vi "Read.vi"(8 "error in (no error)":errorcluster, 9 "timeout (ms)":i32=200, 10 "number to read":i32=100, 11 "CAN RW CANsub in":refnum<class "CAN RW CANsub.lvclass">) -> (0 "error out":errorcluster, 1 "Timeout":bool, 2 "pcap CAN Data":u8[](array[numeric]), 3 "CAN RW CANsub out":refnum<class "CAN RW CANsub.lvclass">, 4 "number read":i32=100)   [LabVIEW 2021, in "CAN RW CANsub.lvclass"]
doc: "Returns pcap CAN packets for at most number to read frames. Reads the socket only when no frames remain from the last read; the socket read waits at most timeout (ms). Applies the allow and deny lists. Timeout is True when no packet is returned and there is no error. Allocates the output array on each call (the interface of CAN_RW_CORE requires it)."
uses:
  CAN RW CANsub.lvclass
  C:/Program Files/National Instruments/LabVIEW 2025/vi.lib/CIF Foundation/CIF CAN RW Core/CAN_RW_CORE.lvclass
  CAN RW CANsub.lvclass/CAN RW CANsub.ctl
  <vilib>/CIF Foundation/CIF CAN RW Core/CAN_RW_CORE.lvclass/CAN_RW_CORE.ctl
  CANsub/c_client/api/CANsub_Channel/CANsub_Channel.lvclass
  CANsub/c_client/api/CANsub_API.lvlib
  <vilib>/CIF Foundation/CIF CAN RW Core/CAN_RW_CORE.lvclass
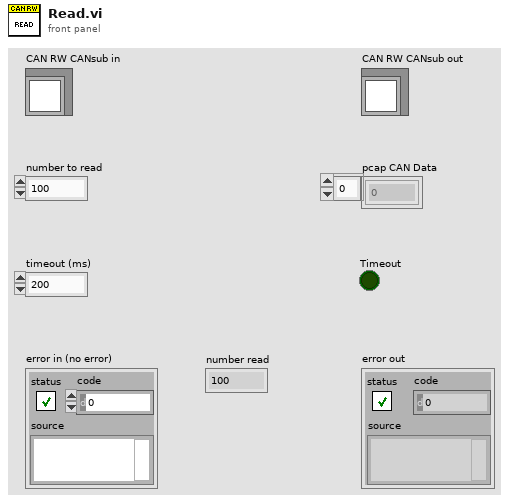
[diagram p1: front panel]
types:
  T1 = typedef "CANsub_API.lvlib/CANsub_Frames.ctl" = cluster{"count":i32, "t_dev":dbl[], "id":u32[], "flags":u16[], "dlc":u8[], "data len":u8[], "data":u8[]}
  T2 = typedef "CANsub_API.lvlib/CANsub_Pcap_Options.ctl" = cluster{"allow list":u32[], "deny list":u32[], "TAI minus UTC (s)":i32, "keep TX acks":bool, "little endian":bool}
  T3 = typedef "CANsub_API.lvlib/CANsub_Pcap_Results.ctl" = cluster{"length":i32, "n packets":i32, "n filtered":i32, "n skipped":i32, "next":i32}
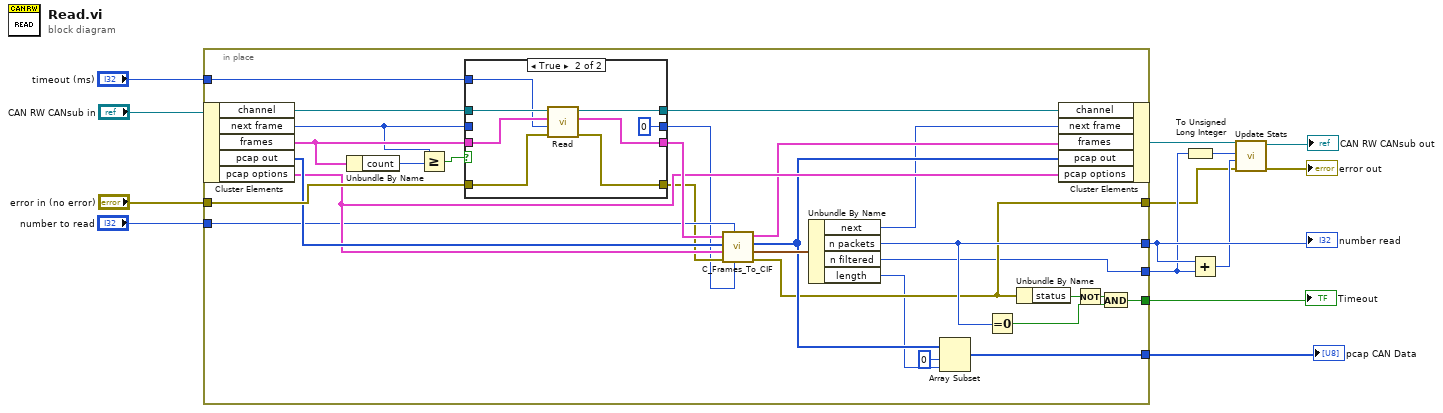
[diagram p0: block diagram]
diagram:
  n1 = in-place {
    in-place-border: [w21] -> w3
    in-place-border: "error in (no error)" -> [w37]
    in-place-border: "number to read" -> [w33]
    in-place-border: "timeout (ms)" -> [w31]
    in-place-border: [w23] -> w10
    in-place-border: [w22] -> w7
    in-place-border: [w18] -> w9
    in-place-border: [w16] -> w5
    n2 = in-place-cluster #1("CAN RW CANsub in") -> ("channel"=w39:refnum<class "CANsub_Channel.lvclass">, "next frame"=w32:i32, "frames"=w38:T1, "pcap out"=w35:u8[], "pcap options"=w34:T2)
    n3 = Unbundle By Name(w38) -> ("count"=w42:i32)
    n4 = Greater Or Equal?(x=w32, y=w42) -> (x >= y?=w41:bool)
    n5 = case shown="True" w41 {
      tunnel: [w46 w53] -> w40
      tunnel: w39 -> [w46 w54]
      tunnel: [w45 0 ("next frame")] -> w27
      tunnel: w32 -> [w45 _]
      tunnel: [w44 w51] -> w36
      tunnel: w38 -> [w44 w52]
      tunnel: [w43 w48] -> w30
      tunnel: w37 -> [w43 w49]
      tunnel: w31 -> [_ w47]
      frame False {
      }
      frame True {
        n6 = call-dynamic "Read.vi"("error in (no error)"=w49, "timeout ms"=w47, "frames in"=w52, "channel in"=w54) -> ("error out"=w48:errorcluster, "frames out"=w51:T1, "channel out"=w53:refnum<class "CANsub_Channel.lvclass">)  [unwired: 5 in]
      }
    }
    n7 = call "C_Frames_To_CIF.vi"("first"=w27, "max packets"=w33, "error in (no error)"=w30, "options"=w34, "pcap in"=w35, "frames in"=w36) -> ("error out"=w21:errorcluster, "result"=w28:T3, "pcap out"=w26:u8[], "frames out"=w29:T1)  [unwired: 2 in]
    n8 = Unbundle By Name(w28) -> ("next"=w24:i32, "n packets"=w22:i32, "n filtered"=w16:i32, "length"=w17:i32)
    n9 = Array Subset(array=w26, index=0, length=w17) -> (w23:u8[])
    n10 = Equal To 0?(x=w22) -> (x = 0?=w19:bool)
    n11 = Unbundle By Name(w21) -> ("status"=w20:bool)
    n12 = in-place-cluster #1("channel"=w40, "next frame"=w24, "frames"=w29, "pcap out"=w26, "pcap options"=w34) -> (w8:refnum<class "CAN RW CANsub.lvclass">)
    n13 = Not(x=w20) -> (.not. x?=w15:bool)
    n14 = And(x=w15, y=w19) -> (x .and. y?=w18:bool)
  }
  "Timeout" <- w9
  "pcap CAN Data" <- w10
  "number read" <- w7
  n15 = To Unsigned Long Integer(number=w5) -> (unsigned 32bit integer=w4:u32)
  n16 = Add(x=w7, y=w5) -> (x+y=w6:i32)
  n17 = call <vilib>:"Update Stats.vi"("error in (no error)"=w3, "Number Read"=w6, "Number Filtered"=w4, "CAN_RW_CORE in"=w8) -> ("error out"=→"error out":errorcluster, "CAN_RW_CORE out"=→"CAN RW CANsub out":refnum<class "CAN RW CANsub.lvclass">)  [unwired: 6 in]
